vi "ERW-IoT Host.vi"   [LabVIEW 2026]
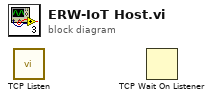
[diagram p0: block diagram]
diagram:
  n1 = call <vilib>:"TCP Listen.vi"() -> ()  [unwired: 7 in, 5 out]
  n2 = TCP Wait On Listener() -> ()  [unwired: 4 in, 5 out]
